vi "Signal Count Assembly.vi"(11 "Long Assembly":bool[][](array[boolean])) -> (0 "S#":i32, 1 "RR#":i32, 2 "Covered?":bool, 3 "Total BC":bool[](array[boolean]), 4 "coverage [%]":dbl, 5 "Total Base CP":i32)   [LabVIEW 2018]
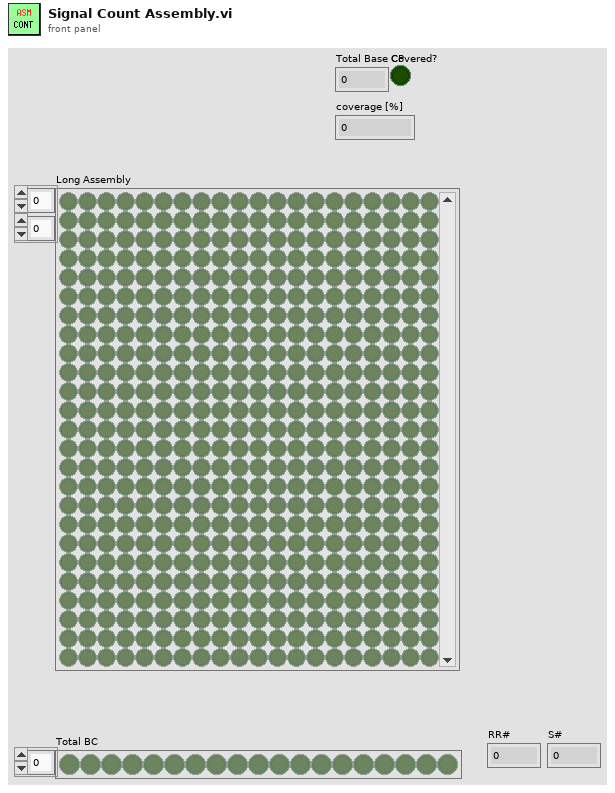
[diagram p1: front panel]
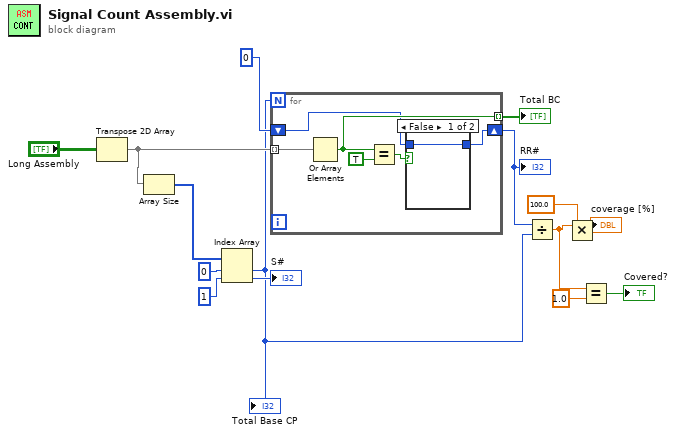
[diagram p0: block diagram]
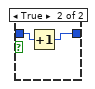
[diagram p2: hidden frame]
diagram:
  n1 = Transpose 2D Array(2D array="Long Assembly") -> (transposed array=w8:bool[][])
  n2 = Array Size(array=w8) -> (size(s)=w15:i32[])
  n3 = Index Array(array=w15, index #1=0 ("Žw•W"), index #2=1 ("Žw•W")) -> (element #1=w6:i32, element #2=→"S#":i32)
  "Total Base CP" <- w6
  n4 = for {
    N: w6 -> [_]
    tunnel: w8 -> [w21] mode=indexing
    tunnel: [w20] -> w12 mode=indexing
    shift-right: [w17] -> w7
    shift-left: 0 -> [w16]
    n5 = Or Array Elements(Boolean array=w21) -> (logical OR=w20:bool)
    n6 = Equal?(x=w20, y=TRUE) -> (x = y?=w18:bool)
    n7 = case shown="False" w18 {
      tunnel: [w22 w24] -> w17
      tunnel: w16 -> [w22 w23]
      frame False {
      }
      frame True {
        n8 = Increment(x=w23) -> (x+1=w24:i32)
      }
    }
  }
  "Total BC" <- w12
  "RR#" <- w7
  n9 = Divide(x=w7, y=w6) -> (x/y=w3:dbl)
  n10 = Multiply(x=w3, y=100.0) -> (x*y=→"coverage [%]":dbl)
  n11 = Equal?(x=w3, y=1.0) -> (x = y?=→"Covered?":bool)
